vi "inline_table_set_sub_table_item.vi"(6 "close_item? (true)":bool=TRUE, 7 "subtables":string[](array[string]), 8 "error in (no error)":errorcluster, 9 "item (value)":refnum<class "Item.lvclass">, 10 "key":string, 11 "InlineTable in":refnum<class "InlineTable.lvclass">) -> (0 "error out":errorcluster, 3 "InlineTable out":refnum<class "InlineTable.lvclass">)   [LabVIEW 2020, in "toml.lvclass"]
uses:
  toml.lvclass
  toml.lvclass/toml.ctl
  InlineTable/InlineTable.lvclass
  Item/Item.lvclass
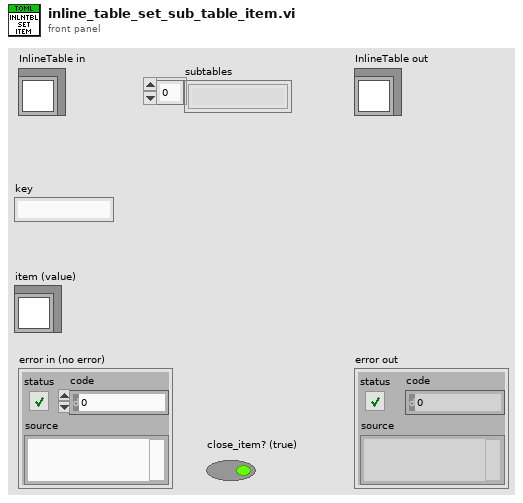
[diagram p1: front panel]
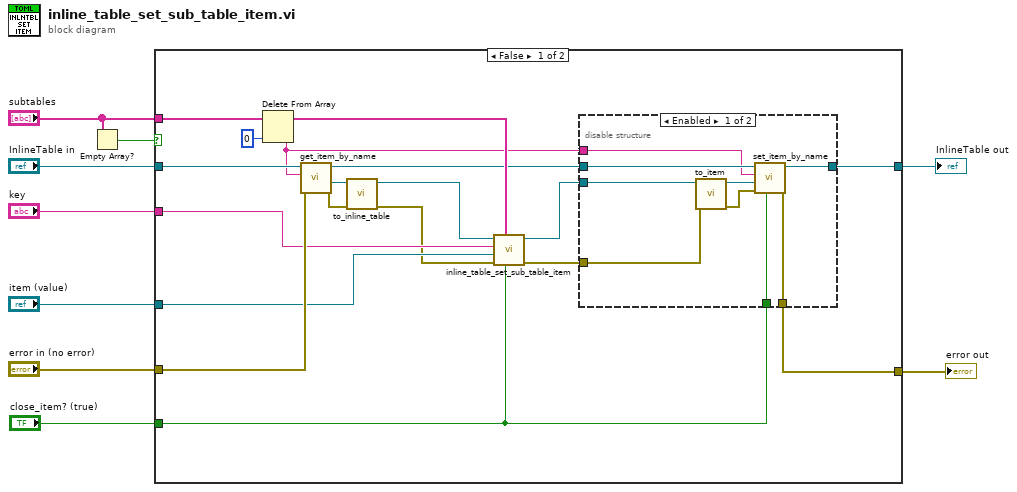
[diagram p0: block diagram]
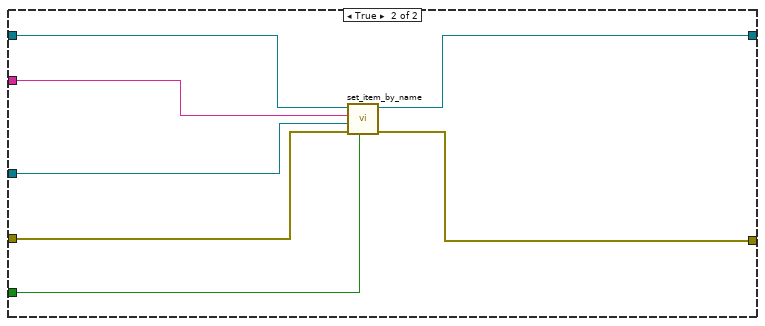
[diagram p3: hidden frame]
diagram:
  n1 = Empty Array?(array="subtables") -> (empty?=w4:bool)
  n2 = case shown="False" w4 {
    tunnel: [w20 w45] -> w9
    tunnel: "item (value)" -> [w21 w42]
    tunnel: [w16 w44] -> w7
    tunnel: "InlineTable in" -> [w24 w43]
    tunnel: "error in (no error)" -> [w23 w41]
    tunnel: "subtables" -> [w27 _]
    tunnel: "close_item? (true)" -> [w14 w40]
    tunnel: "key" -> [w15 w39]
    frame False {
      n3 = Delete From Array(array=w27, index=0) -> (deleted portion=w19:string, array with subset deleted=w25:string[])  [unwired: 1 in]
      n4 = call "get_item_by_name.vi"("error in (no error)"=w23, "key_name"=w19, "Table in"=w24) -> ("error out"=w13:errorcluster, "Item"=w12:refnum<class "Item.lvclass">, "Table out"=w22:refnum<class "InlineTable.lvclass">)  [unwired: 6 in]
      n5 = call "to_inline_table.vi"("error in (no error)"=w13, "Item in"=w12) -> ("error out"=w10:errorcluster, "InlineTable"=w11:refnum<class "InlineTable.lvclass">)  [unwired: 8 in]
      n6 = call "inline_table_set_sub_table_item.vi"("close_item? (true)"=w14, "subtables"=w25, "error in (no error)"=w10, "item (value)"=w21, "key"=w15, "InlineTable in"=w11) -> ("error out"=w17:errorcluster, "InlineTable out"=w18:refnum<class "InlineTable.lvclass">)  [unwired: 4 in]
      n7 = disable-structure shown="Enabled" {
        disable-tunnel: w22 -> [w36 w38]
        disable-tunnel: [w35 w37] -> w20
        disable-tunnel: w19 -> [w34 _]
        disable-tunnel: w18 -> [w33 _]
        disable-tunnel: w17 -> [w32 w37]
        disable-tunnel: [w30 w38] -> w16
        disable-tunnel: w14 -> [w29 _]
        frame Enabled {
          n8 = call "to_item.vi"("error in (no error)"=w32, "Table in"=w33) -> ("error out"=w31:errorcluster, "Item out"=w28:refnum<class "Item.lvclass">)  [unwired: 8 in]
          n9 = call "set_item_by_name.vi"("close_item? (true)"=w29, "error in"=w31, "Item"=w28, "key_name"=w34, "Table in"=w36) -> ("error out"=w35:errorcluster, "Table out"=w30:refnum<class "InlineTable.lvclass">)  [unwired: 5 in]
        }
        frame Disabled {
        }
      }
    }
    frame True {
      n10 = call "set_item_by_name.vi"("close_item? (true)"=w40, "error in"=w41, "Item"=w42, "key_name"=w39, "Table in"=w43) -> ("error out"=w45:errorcluster, "Table out"=w44:refnum<class "InlineTable.lvclass">)  [unwired: 5 in]
    }
  }
  "error out" <- w9
  "InlineTable out" <- w7
